vi "clone.vi"(0 "reference in":refnum<class "DQMHModuleNode.lvclass">, 5 "error in (no error)":errorcluster) -> (14 "reference out":refnum<class "DQMHModuleNode.lvclass">, 15 "clonedClassNode":refnum<class "AbstractNode.lvclass">, 19 "error out":errorcluster)   [LabVIEW 2020, in "DQMHModuleNode.lvclass"]
doc: "public Object clone()"
uses:
  <resource>/Framework/Providers/Open_GDS/UML/DQMHModuleNode_class/DQMHModuleNode.lvclass
  C:/Program Files (x86)/National Instruments/LabVIEW 2020/resource/Framework/Providers/Open_GDS/UML/RectangularNode_class/RectangularNode.lvclass
  C:/Program Files (x86)/National Instruments/LabVIEW 2020/resource/Framework/Providers/Open_GDS/UML/AbstractNode_class/AbstractNode.lvclass
  <resource>/Framework/Providers/Open_GDS/UML/AbstractNode_class/AbstractNode.lvclass
  <resource>/Framework/Providers/Open_GDS/UML/MultiLineString_class/MultiLineString.lvclass
  <resource>/Framework/Providers/Open_GDS/UML/RectangularNode_class/RectangularNode.lvclass
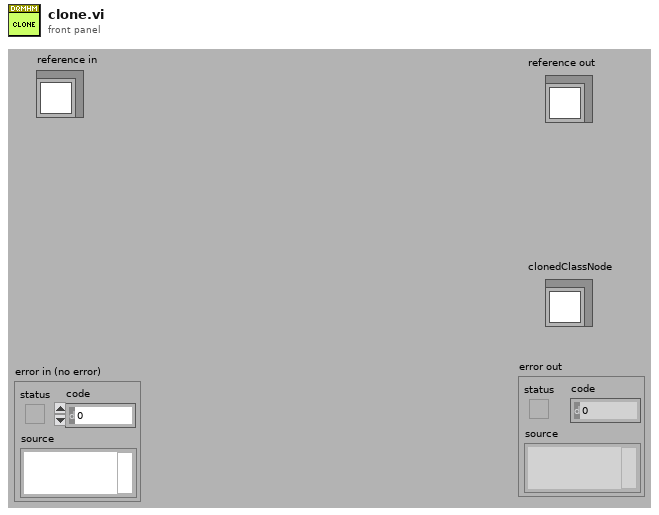
[diagram p1: front panel]
types:
  T1 = typedef "RectangularNode.lvclass/ObjectAttributes.ctl" = cluster{"bounds":T2}
  T2 = typedef "Rectangle Rectangle2D.ctl" = cluster{"x":dbl, "y":dbl, "width":dbl, "height":dbl}
  T3 = typedef "DQMHModuleNode.lvclass/ObjectAttributes.ctl" = cluster{"DescriptionHeight":dbl, "InternalDataHeight":dbl, "EventsHeight":dbl, "Name":refnum<class "MultiLineString.lvclass">, "Description":refnum<class "MultiLineString.lvclass">, "InternalData":refnum<class "MultiLineString.lvclass">, "Events":refnum<class "MultiLineString.lvclass">, "showDescription":bool, "showInternalData":bool, "showEvents":bool, "DEFAULT_ROUNDING":i32, "DEFAULT_WIDTH":i32, "DEFAULT_HEIGHT":i32, "ClassPath":path, "Template":string, "Icon":u8[][]}
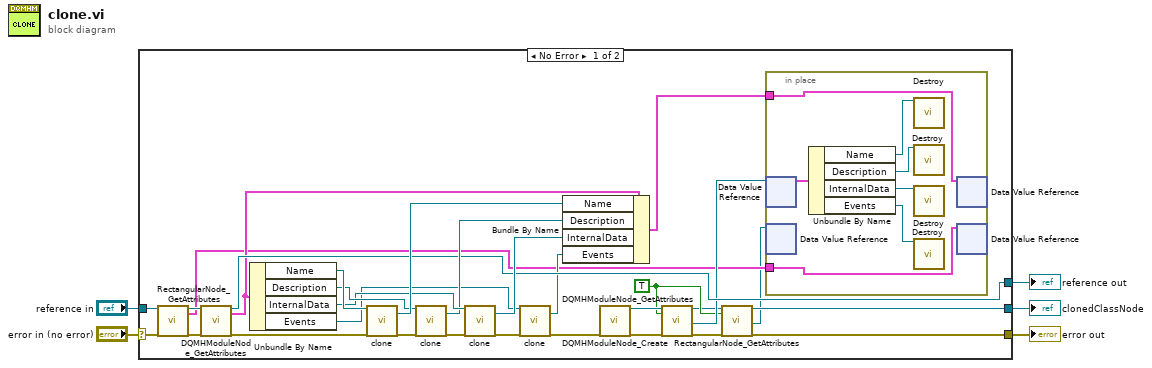
[diagram p0: block diagram]
diagram:
  n1 = case shown="No Error" "error in (no error)" {
    selector: "error in (no error)" -> [w16 w43]
    tunnel: "reference in" -> [w15 w44]
    tunnel: [w7 w43] -> w4
    tunnel: [w24 w44] -> w3
    tunnel: [w8 _] -> w1
    frame No Error {
      w11 = TRUE ("OnlyGetDvrReference(False)")
      n2 = call <resource>:"RectangularNode_GetAttributes.vi"("reference in"=w15, "error in (no error)"=w16) -> ("reference out"=w14:refnum<class "DQMHModuleNode.lvclass">, "Data"=w12:T1, "error out"=w13:errorcluster)  [unwired: 14 in, 1 out]
      n3 = call <resource>:"DQMHModuleNode_GetAttributes.vi"("reference in"=w14, "error in (no error)"=w13) -> ("reference out"=w24:refnum<class "DQMHModuleNode.lvclass">, "Data"=w23:T3, "error out"=w27:errorcluster)  [unwired: 1 in, 14 out]
      n4 = Unbundle By Name(w23) -> ("Name"=w35:refnum<class "MultiLineString.lvclass">, "Description"=w31:refnum<class "MultiLineString.lvclass">, "InternalData"=w30:refnum<class "MultiLineString.lvclass">, "Events"=w20:refnum<class "MultiLineString.lvclass">)
      n5 = call-dynamic "clone.vi"("reference"=w35, "error in (no error)"=w27) -> ("clonedMultiLineString"=w34:refnum<class "MultiLineString.lvclass">, "error out"=w33:errorcluster)  [unwired: 15 in, 1 out]
      n6 = call-dynamic "clone.vi"("reference"=w31, "error in (no error)"=w33) -> ("clonedMultiLineString"=w29:refnum<class "MultiLineString.lvclass">, "error out"=w32:errorcluster)  [unwired: 15 in, 1 out]
      n7 = call-dynamic "clone.vi"("reference"=w30, "error in (no error)"=w32) -> ("clonedMultiLineString"=w28:refnum<class "MultiLineString.lvclass">, "error out"=w19:errorcluster)  [unwired: 15 in, 1 out]
      n8 = call-dynamic "clone.vi"("reference"=w20, "error in (no error)"=w19) -> ("clonedMultiLineString"=w17:refnum<class "MultiLineString.lvclass">, "error out"=w18:errorcluster)  [unwired: 15 in, 1 out]
      n9 = Bundle By Name(cluster=w23, "Name"=w34, "Description"=w29, "InternalData"=w28, "Events"=w17) -> (w21:T3)
      n10 = call <resource>:"DQMHModuleNode_Create.vi"("error in (no error)"=w18) -> ("reference out"=w26:refnum<class "DQMHModuleNode.lvclass">, "error out"=w25:errorcluster)  [unwired: 17 in]
      n11 = call <resource>:"DQMHModuleNode_GetAttributes.vi"("reference in"=w26, "OnlyGetDvrReference(False)"=w11, "error in (no error)"=w25) -> ("reference out"=w10:refnum<class "DQMHModuleNode.lvclass">, "DataRef"=w22:refnum<data-value>, "error out"=w9:errorcluster)  [unwired: 13 in, 1 out]
      n12 = call <resource>:"RectangularNode_GetAttributes.vi"("reference in"=w10, "OnlyGetDvrReference(False)"=w11, "error in (no error)"=w9) -> ("reference out"=w8:refnum<class "DQMHModuleNode.lvclass">, "DataRef"=w6:refnum<data-value>, "error out"=w7:errorcluster)  [unwired: 13 in, 1 out]
      n13 = in-place {
        in-place-border: w21 -> [w42]
        in-place-border: w12 -> [w36]
        n14 = in-place-dvr #1(w22) -> (w41:T3)  [unwired: 1 out]
        n15 = in-place-dvr #2(w6) -> ()  [unwired: 2 out]
        n16 = Unbundle By Name(w41) -> ("Name"=w40:refnum<class "MultiLineString.lvclass">, "Description"=w39:refnum<class "MultiLineString.lvclass">, "InternalData"=w38:refnum<class "MultiLineString.lvclass">, "Events"=w37:refnum<class "MultiLineString.lvclass">)
        n17 = call-dynamic "Destroy.vi"("reference"=w40) -> ()  [unwired: 17 in, 2 out]
        n18 = call-dynamic "Destroy.vi"("reference"=w39) -> ()  [unwired: 17 in, 2 out]
        n19 = call-dynamic "Destroy.vi"("reference"=w38) -> ()  [unwired: 17 in, 2 out]
        n20 = call-dynamic "Destroy.vi"("reference"=w37) -> ()  [unwired: 17 in, 2 out]
        n21 = in-place-dvr #1(w42) -> ()  [unwired: 2 out]
        n22 = in-place-dvr #2(w36) -> ()  [unwired: 2 out]
      }
    }
    frame Error {
    }
  }
  "reference out" <- w3
  "error out" <- w4
  "clonedClassNode" <- w1
